vi "All 1.vi"() -> ()   [LabVIEW 2020, in "Benchmark.lvlib"]
uses:
  Benchmark.lvlib
  <vilib>/Analysis/NI_AALBase.lvlib
  Main/Scene/Scene.lvclass
  Libraries/Utility/Utility.lvlib
panel:
  out "2D Picture":picture
  out "Mean FPS":dbl format="%.1p"
  out "Std Dev":dbl format="%.1p"
  out "Mean":dbl format="%.1p"
  out "Histogram Graph":T1(graph)
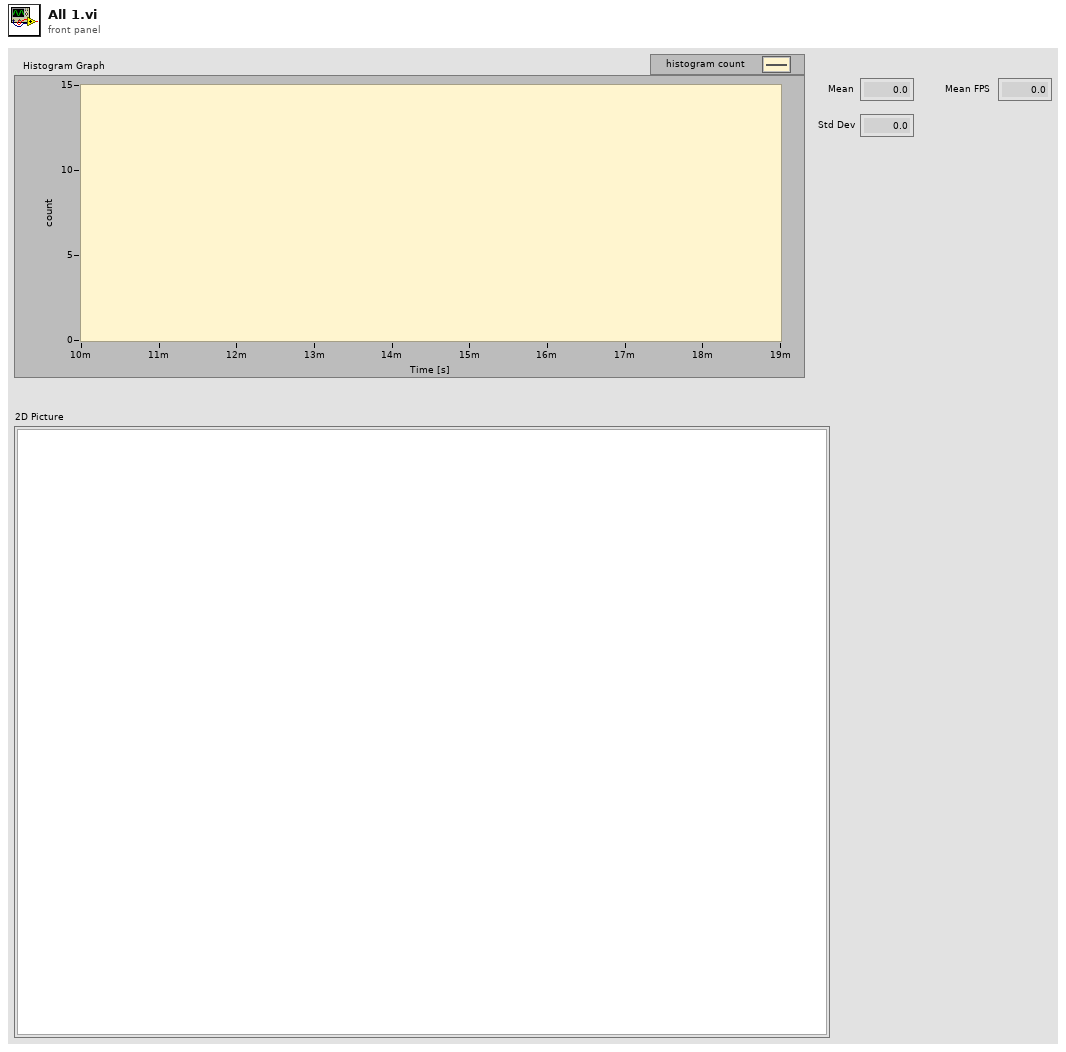
[diagram p1: front panel]
types:
  T1 = cluster{"X Values":dbl[], "Histogram: h(x)":i32[]}
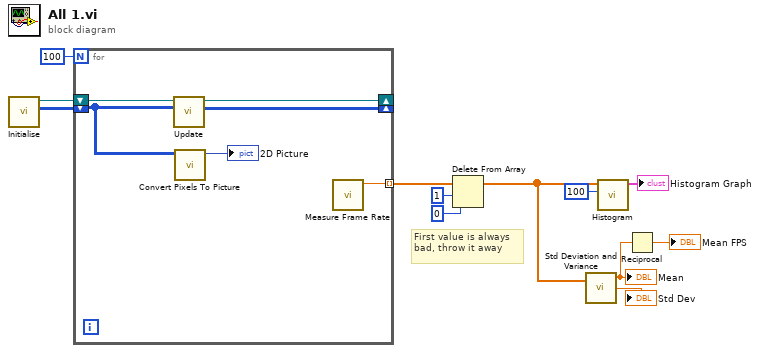
[diagram p0: block diagram]
diagram:
  # "First value is always bad, throw it away"
  n1 = call "Initialise.vi"() -> ("Pixel Data out"=w7:u32[][], "Scene out"=w8:refnum<class "Scene.lvclass">)  [unwired: 10 in]
  n2 = for {
    N: 100 -> [_]
    tunnel: [w13] -> w4 mode=indexing
    shift-right: [w15] -> _
    shift-left: w7 -> [w18]
    shift-right: [w14] -> _
    shift-left: w8 -> [w17]
    n3 = call "Update.vi"("Pixel Data in"=w18, "Scene in"=w17) -> ("Pixel Data out"=w15:u32[][], "Scene out"=w14:refnum<class "Scene.lvclass">)  [unwired: 8 in]
    n4 = call "Convert Pixels To Picture.vi"("Pixel Data in"=w18) -> ("2D Picture"=→"2D Picture":picture)  [unwired: 9 in, 1 out]
    n5 = call "Measure Frame Rate.vi"() -> ("Delta Time [s]"=w13:dbl)  [unwired: 10 in, 1 out]
  }
  n6 = Delete From Array(array=w4, length=1, index=0) -> (array with subset deleted=w3:dbl[])  [unwired: 1 out]
  n7 = call <vilib>:"Std Deviation and Variance.vi"("X"=w3) -> ("mean"=w6:dbl, "standard deviation"=→"Std Dev":dbl)  [unwired: 1 in, 1 out]
  "Mean" <- w6
  n8 = call <vilib>:"Histogram.vi"("intervals"=100, "X"=w3) -> ("Histogram Graph"=→"Histogram Graph":T1)  [unwired: 6 in, 3 out]
  n9 = Reciprocal(x=w6) -> (1/x=→"Mean FPS":dbl)
